vi "AuthService SubscribeLogin Read.vi"(8 "error in":errorcluster, 11 "Call ID in":T3) -> (0 "error out":errorcluster, 1 "Success":bool, 2 "Response Data":T1, 3 "Call ID":T3)   [LabVIEW 2020, in "grpc-auth_client.lvlib"]
uses:
  grpc-auth_client.lvlib
  <vilib>/gRPC/LabVIEW gRPC Library/Shared/grpcId.ctl
  RPC Messages/auth_SubscribeLoginResponse.ctl
  RPC Messages/auth_LoginStatus.ctl
  RPC Messages/auth_SubscribeLoginResponse_Flat.ctl
  aea5dbbb-03a2-479b-ad95-94da4ee1cea9.vi
  <vilib>/gRPC/LabVIEW gRPC Library/Shared/TranslateGrpcError.vi
  <vilib>/gRPC/LabVIEW gRPC Library/Shared/Wait On Occurrence.vi
  <vilib>/gRPC/LabVIEW gRPC Library/Shared/Is Feature Enabled.vi
  <vilib>/gRPC/LabVIEW gRPC Library/Server API/Server/Get Server DLL Path.vi
  <vilib>/Utility/error.llb/Error Cluster From Error Code.vi
  <vilib>/gRPC/LabVIEW gRPC Library/grpc-lvsupport-release.lvlib
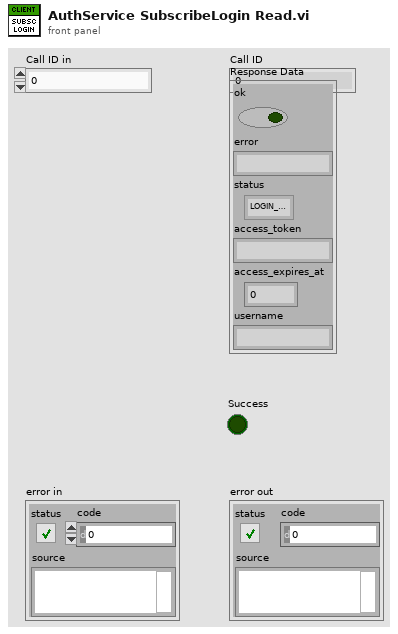
[diagram p1: front panel]
types:
  T1 = typedef "grpc-auth_client.lvlib/auth_SubscribeLoginResponse.ctl" = cluster{"ok":bool, "error":string, "status":T2, "access_token":string, "access_expires_at":i64, "username":string}
  T2 = typedef "grpc-auth_client.lvlib/auth_LoginStatus.ctl" = enum32{"LOGIN_STATUS_PENDING", "LOGIN_STATUS_READY", "LOGIN_STATUS_EXPIRED", "LOGIN_STATUS_USED", "LOGIN_STATUS_INVALID"}
  T3 = typedef "grpc-lvsupport-release.lvlib/grpcId.ctl" = u64
  T4 = typedef "grpc-auth_client.lvlib/auth_SubscribeLoginResponse_Flat.ctl" = cluster{"ok":bool, "error":string, "status":T2, "access_token":string, "access_expires_at":i64, "username":string}
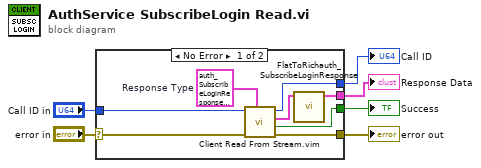
[diagram p0: block diagram]
diagram:
  n1 = case shown="No Error" "error in" {
    selector: "error in" -> [w14 w15]
    tunnel: [w13 w15] -> w5
    tunnel: "Call ID in" -> [w12 w16]
    tunnel: [w10 w16] -> w3
    tunnel: [w7 _] -> w2
    tunnel: [w11 _] -> w1
    frame No Error {
      w9 = T4 {"ok"=FALSE, "error"="", "status"=enum."LOGIN_STATUS_PENDING", "access_token"="", "access_expires_at"=0, "username"=""}  # Response Type
      n2 = call "Client Read From Stream.vim"("Response Type"=w9, "error in"=w14, "Call ID in"=w12) -> ("error out"=w13:errorcluster, "Success"=w11:bool, "Response Data"=w8:T4, "Call ID out"=w10:u64)  [unwired: 5 in]
      n3 = call "FlatToRichauth_SubscribeLoginResponse.vi"("InputCluster"=w8) -> ("OutputCluster"=w7:T1)  [unwired: 10 in]
    }
    frame Error {
    }
  }
  "error out" <- w5
  "Call ID" <- w3
  "Response Data" <- w2
  "Success" <- w1
